vi "TemplatePanel_Child.vi"(7 "Set(F)":bool, 8 "error in (no error)":errorcluster, 10 "First Time(F)":bool, 11 "object in":refnum<class>) -> (0 "error out":errorcluster, 2 "Changed?":bool, 3 "object out":refnum<class>)   [LabVIEW 2021, in "Template-ChannelsChild.lvlib" / "Template_CFG.lvclass"]
uses:
  Template_CFG.lvclass
  tdef/Data.ctl
  Template_CFG.lvclass/Template_CFG.ctl
panel:
  in  "Save Button":bool
  in  "TemplateData":T1
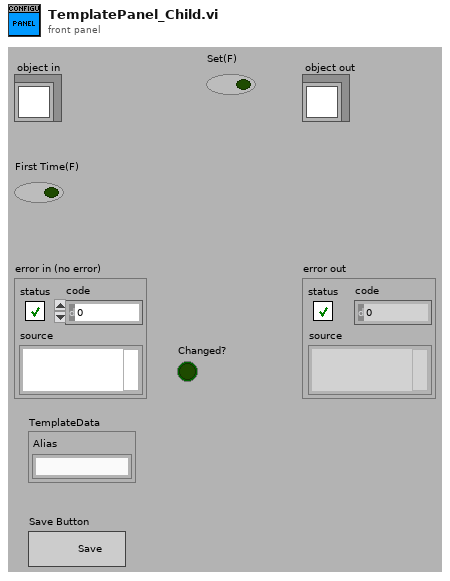
[diagram p1: front panel]
types:
  T1 = typedef "Template-ChannelsChild.lvlib/Template_CFG.lvclass/Data.ctl" = cluster{"Alias":string}
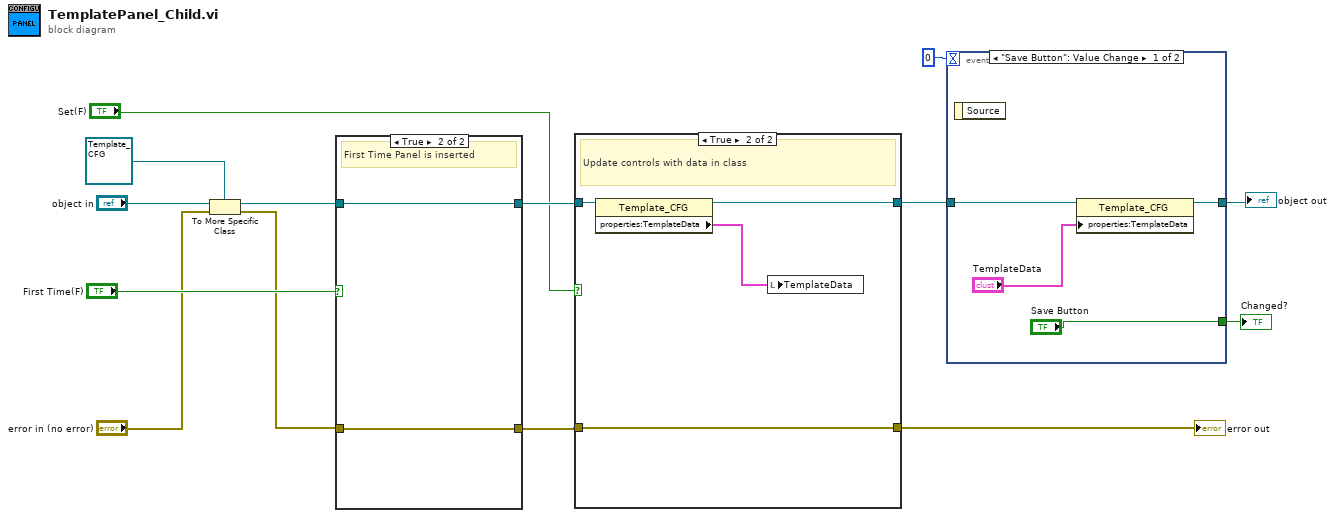
[diagram p0: block diagram]
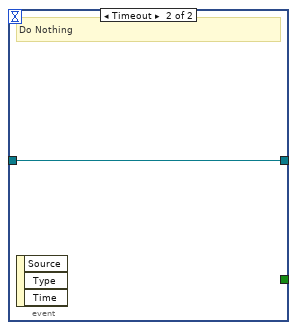
[diagram p2: hidden frame]
diagram:
  n1 = To More Specific Class(target class=refnum<class "Template_CFG.lvclass"> refnum ("Template-Channels.lvlib:Template_CFG"), reference="object in", error in="error in (no error)") -> (specific class reference=w8:refnum<class "Template_CFG.lvclass">, error out=w6:errorcluster)
  n2 = case shown="True" "First Time(F)" {
    tunnel: [w16 w18] -> w12
    tunnel: w8 -> [w16 w18]
    tunnel: [w15 w17] -> w11
    tunnel: w6 -> [w15 w17]
    frame False {
    }
    frame True {
      # "First Time Panel is inserted"
    }
  }
  n3 = case shown="True" "Set(F)" {
    tunnel: [w20 w22] -> w3
    tunnel: w12 -> [w20 w24]
    tunnel: [w19 w23] -> w10
    tunnel: w11 -> [w19 w23]
    frame False {
    }
    frame True {
      # "Update controls with data in class"
      n4 = property class="Template_CFG"(reference=w24) -> (reference out=w22:refnum<class "Template_CFG.lvclass">, "properties:TemplateData"=w21:T1)  [unwired: 1 in, 1 out]
      n5 = local write "TemplateData"(w21) -> ()
    }
  }
  "error out" <- w10
  n6 = event shown="[0] \"Save Button\": Value Change" {
    selector: _ -> [_ _]
    dyn-events: _ -> [_ _]
    timeout: 0 -> [_ _]
    tunnel: [w28 w29] -> w4
    tunnel: w3 -> [w27 w29]
    tunnel: ["Save Button" _] -> w1
    event "Save Button": Value Change {
      n7 = event-data() -> ()  [unwired: 1 in, 1 out]
      n8 = property class="Template_CFG"(reference=w27, "properties:TemplateData"="TemplateData") -> (reference out=w28:refnum<class "Template_CFG.lvclass">)  [unwired: 1 in, 1 out]
    }
    event Timeout {
      # "Do Nothing"
      n9 = event-data() -> ()  [unwired: 1 in, 3 out]
    }
  }
  "object out" <- w4
  "Changed?" <- w1
